vi "Func - Load FuncVI & test arg num.vi"(5 "test arg num":bool, 6 "error in":errorcluster, 8 "arg num":i32, 9 "func name":string) -> (0 "error out":errorcluster, 1 "error message":string, 3 "FuncVI RefNum":refnum<vi>, 4 "loaded":bool)   [LabVIEW 2021]
doc: "::: CalcExpress Toolkit :::\nCopyright (c) 2000-2026 Konstantin Shifershteyn. All rights reserved."
panel:
  in  "VI Refnum":refnum<vi>
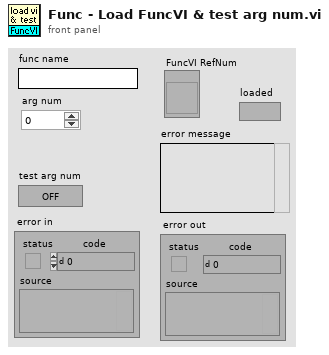
[diagram p1: front panel]
types:
  T1 = cluster{"open to call":bool, "Enable FuncVI2":bool}
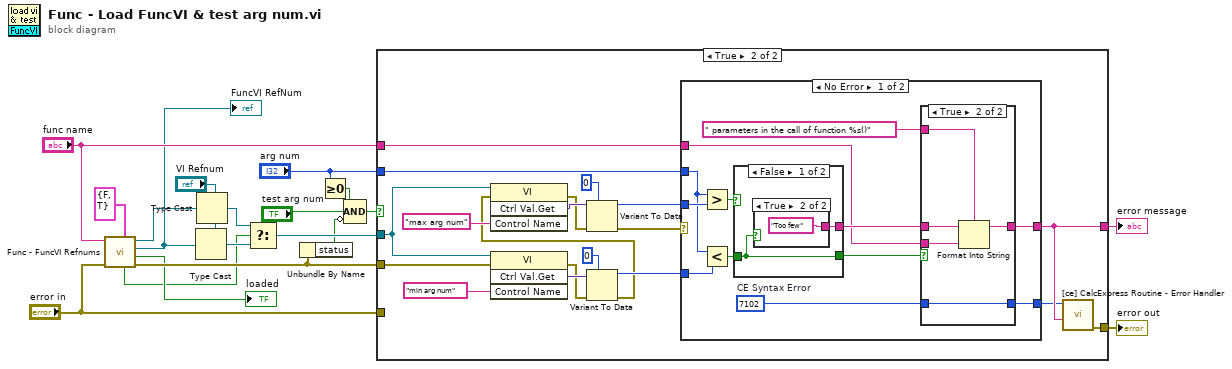
[diagram p0: block diagram]
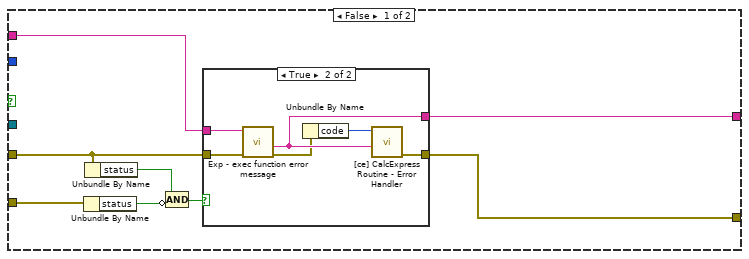
[diagram p2: hidden frame]
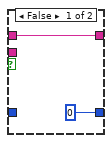
[diagram p4: hidden frame]
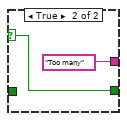
[diagram p6: hidden frame]
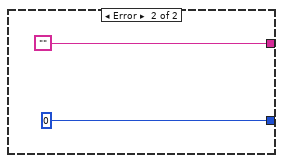
[diagram p7: hidden frame]
diagram:
  n1 = call "Func - FuncVI Refnums.vi"("Params"=T1 {"open to call"=FALSE, "Enable FuncVI2"=TRUE}, "error in"="error in", "Func name"="func name") -> ("error out"=w19:errorcluster, "loaded"=→"loaded":bool, "FuncVI RefNum out"=w4:refnum<vi>, "FuncVI2 RefNum out"=w6:refnum<vi>, "FuncVI2"=w3:bool)  [unwired: 4 in]
  "FuncVI RefNum" <- w4
  n2 = Type Cast(type="VI Refnum", x=w4) -> (*(type *) &x=w10:refnum<vi>)
  n3 = Type Cast(type="VI Refnum", x=w6) -> (*(type *) &x=w9:refnum<vi>)
  n4 = Select(t=w9, s=w3, f=w10) -> (s? t:f=w8:refnum<vi>)
  n5 = Unbundle By Name(w19) -> ("status"=w7:bool)
  n6 = Greater Or Equal To 0?(x="arg num") -> (x >= 0?=w17:bool)
  n7 = Compound Arithmetic op=AND(w17, "test arg num", invert w7) -> (w16:bool)
  n8 = case shown="True" w16 {
    tunnel: w19 -> [w21 w47]
    tunnel: w8 -> [_ w46]
    tunnel: "error in" -> [w27 _]
    tunnel: "arg num" -> [_ w52]
    tunnel: "func name" -> [w25 w51]
    tunnel: [w23 w50] -> w12
    tunnel: [w22 w49] -> w13
    frame False {
      n9 = Unbundle By Name(w27) -> ("status"=w26:bool)
      n10 = Unbundle By Name(w21) -> ("status"=w20:bool)
      n11 = Compound Arithmetic op=AND(w20, invert w26) -> (w24:bool)
      n12 = case shown="True" w24 {
        tunnel: w21 -> [w28 w34]
        tunnel: w25 -> [_ w33]
        tunnel: [w28 w29] -> w23
        tunnel: [_ w32] -> w22
        frame False {
        }
        frame True {
          n13 = call "Exp - exec function error message.vi"("error in"=w34, "func name"=w33) -> ("error out"=w30:errorcluster, "error message"=w32:string)  [unwired: 6 in]
          n14 = Unbundle By Name(w30) -> ("code"=w31:i32)
          n15 = call "[ce] CalcExpress Routine - Error Handler.vi"("error msg"=w32, "error code"=w31) -> ("error out"=w29:errorcluster)  [unwired: 7 in]
        }
      }
    }
    frame True {
      n16 = invoke on="Invoke Node" class="VI" method="Ctrl Val.Get"(reference=w46, error in=w47, "Control Name"="min arg num") -> (error out=w38:errorcluster, "Get Control Value Variant"=w40:variant)  [unwired: 1 in, 2 out]
      n17 = Variant To Data(error in=w38, type=0, Variant=w40) -> (data=w37:i32, error out=w36:errorcluster)
      n18 = invoke on="Invoke Node" class="VI" method="Ctrl Val.Get"(reference=w46, error in=w36, "Control Name"="max arg num") -> (error out=w44:errorcluster, "Get Control Value Variant"=w45:variant)  [unwired: 1 in, 2 out]
      n19 = Variant To Data(error in=w44, type=0, Variant=w45) -> (data=w42:i32, error out=w35:errorcluster)
      n20 = case shown="No Error" w35 {
        tunnel: w37 -> [w64 _]
        tunnel: w42 -> [w65 _]
        tunnel: [w59 "" ("Empty String Constant")] -> w49
        tunnel: w52 -> [w57 _]
        tunnel: w51 -> [w56 _]
        tunnel: [w55 0 ("CE Syntax Error")] -> w48
        frame No Error {
          w54 = 7102  # CE Syntax Error
          n21 = Greater?(x=w57, y=w65) -> (0:w63:bool)
          n22 = Less?(x=w57, y=w64) -> (x < y?=w62:bool)
          n23 = case shown="False" w63 {
            selector: w63 -> [_ w77]
            tunnel: w62 -> [w73 _]
            tunnel: [w74 "Too many"] -> w60
            tunnel: [w73 w77] -> w58
            frame False {
              n24 = case shown="True" w73 {
                tunnel: [_ "Too few"] -> w74
                frame False {
                }
                frame True {
                }
              }
            }
            frame True {
            }
          }
          n25 = case shown="True" w58 {
            tunnel: " parameters in the call of function %s()" -> [_ w72]
            tunnel: w60 -> [w67 w71]
            tunnel: [w67 w70] -> w59
            tunnel: w56 -> [_ w69]
            tunnel: [0 w68] -> w55
            tunnel: w54 -> [_ w68]
            frame False {
            }
            frame True {
              n26 = Format Into String(format string=w72, initial string=w71, w69) -> (resulting string=w70:string)  [unwired: 1 in, 1 out]
            }
          }
        }
        frame Error {
        }
      }
      n27 = call "[ce] CalcExpress Routine - Error Handler.vi"("error msg"=w49, "error code"=w48) -> ("error out"=w50:errorcluster)  [unwired: 7 in]
    }
  }
  "error out" <- w12
  "error message" <- w13
